vi "LC_Read_Number.vi"(8 "Cutted Sample Sequence":string="TCTAGACTATCTCACTCTCAGATGAGATCGATAGATCAGT", 9 "Level Composition":string[](array[string]), 11 "LSPX_C2":T1) -> (3 "Assigned#_CL":T2)   [LabVIEW 2018]
panel:
  out "Tri_MxRight#":i32[](array[numeric])
  out "Di_MxRight#":i32[](array[numeric])
  out "Mono_MxRight#":i32[](array[numeric])
  out "Tri_Assigned#":i32[](array[numeric])
  out "Di_Assigned#":i32[](array[numeric])
  out "Mono_Assigned#":i32[](array[numeric])
  out "MxRight_Array":string[](array[string])
  out "Assigned_Array":string[](array[string])
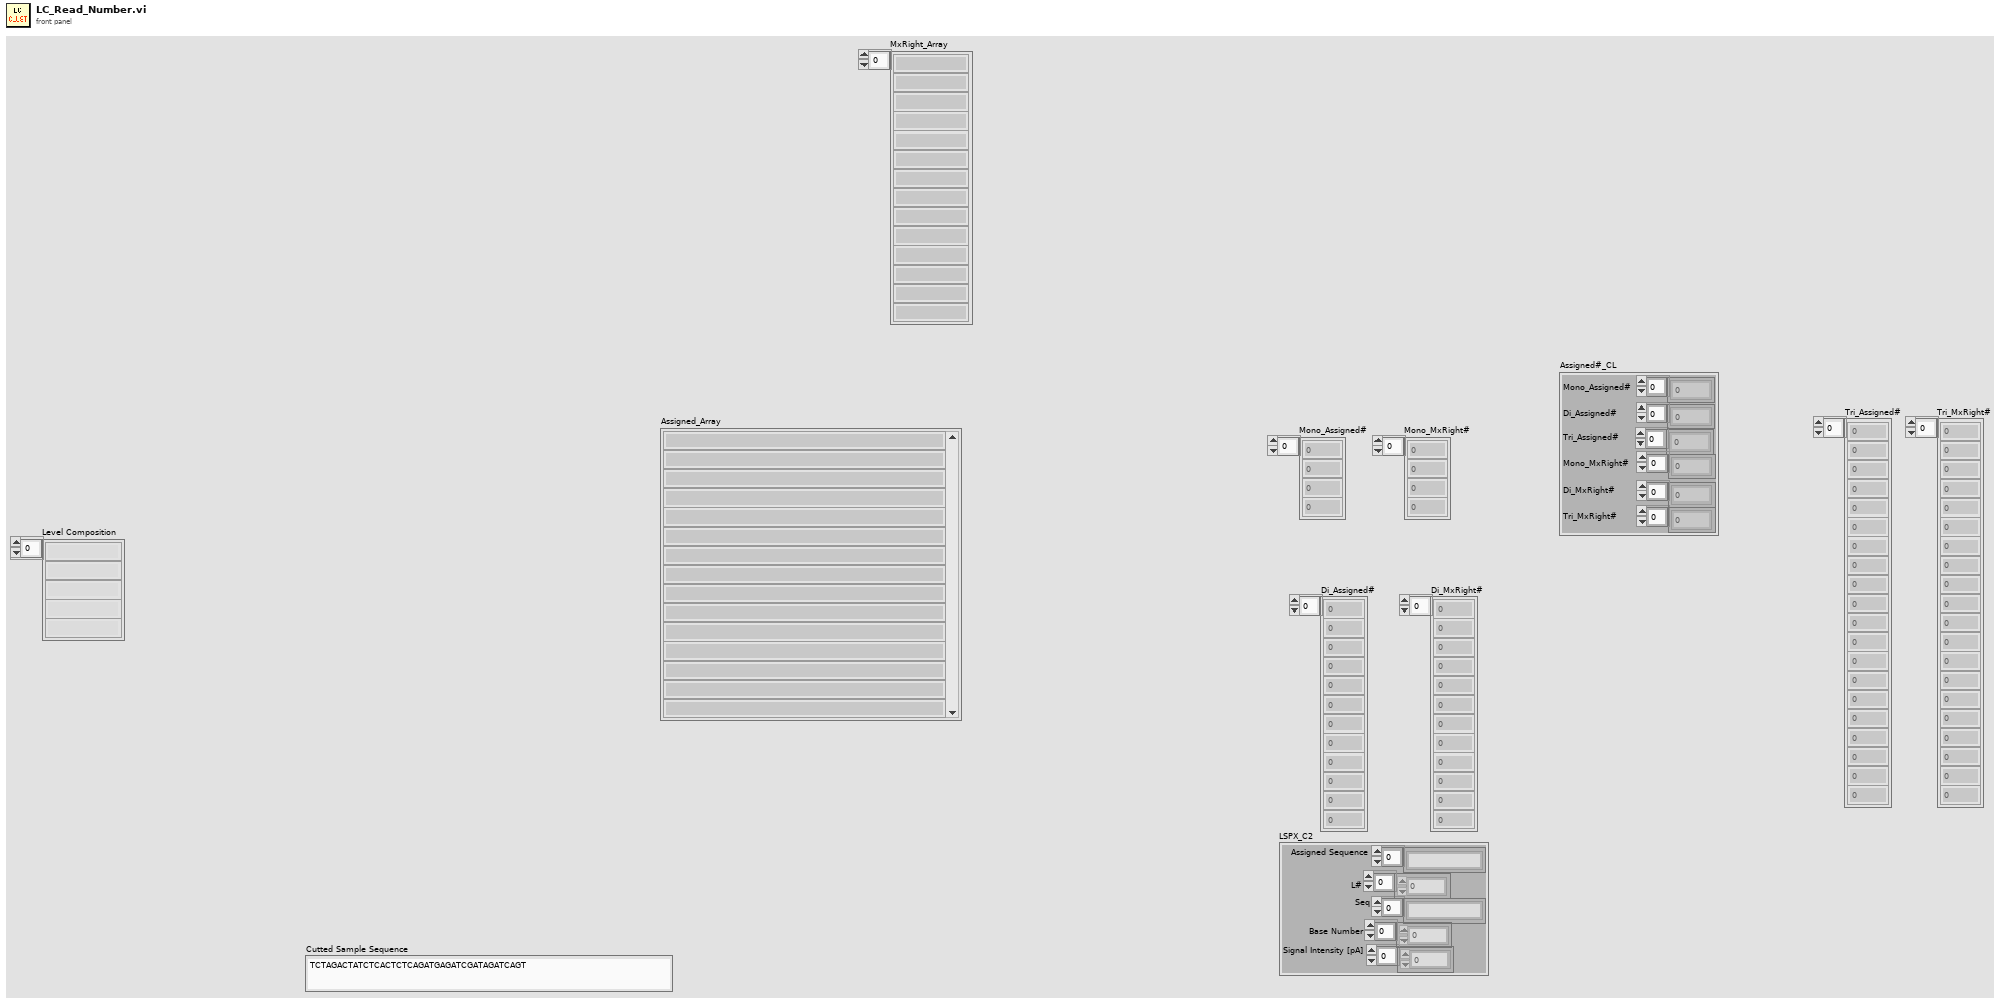
[diagram p1: front panel]
types:
  T1 = cluster{"Assigned Sequence":string[], "L#":i32[], "Seq":string[], "Base Number":i32[], "Signal Intensity [pA]":dbl[]}
  T2 = cluster{"Mono_Assigned#":i32[], "Di_Assigned#":i32[], "Tri_Assigned#":i32[], "Tri_MxRight#":i32[], "Di_MxRight#":i32[], "Mono_MxRight#":i32[]}
  T3 = cluster{"MonoBase_Array_Tag":string[], "DiBase_Array_Tag":string[], "TriBase_Array_Tag":string[]}
  T4 = cluster{i32[], i32[], i32[], i32[], i32[], i32[]}
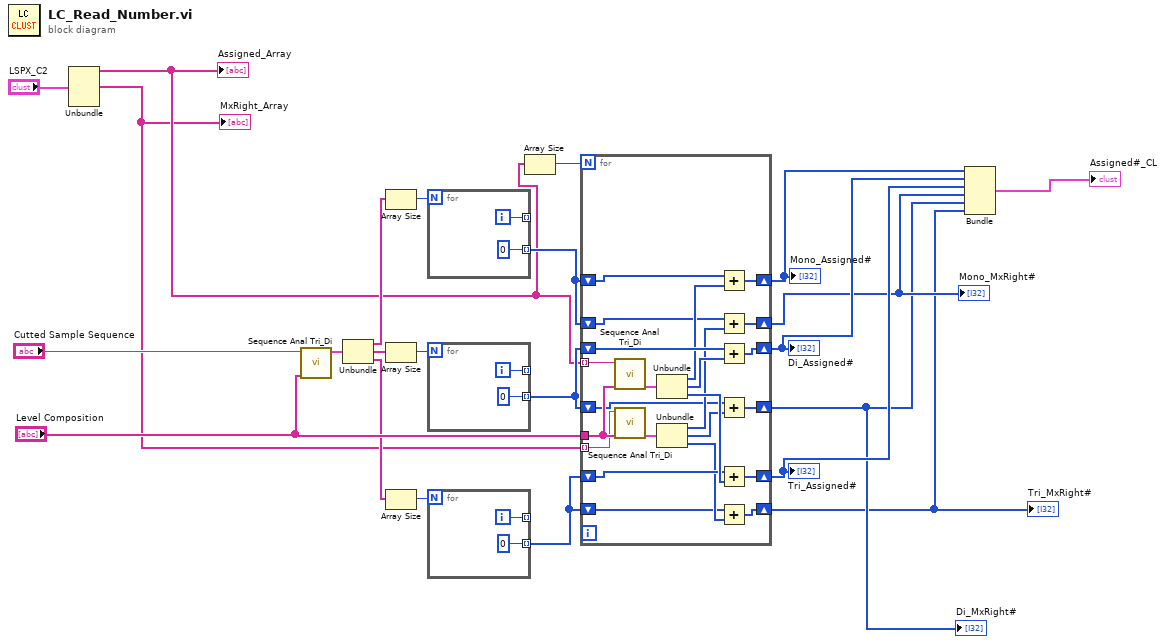
[diagram p0: block diagram]
diagram:
  n1 = Unbundle("LSPX_C2") -> ("Assigned Sequence"=w5:string[], "Seq"=w4:string[])  [unwired: 3 out]
  "Assigned_Array" <- w5
  "MxRight_Array" <- w4
  n2 = call "Sequence Anal Tri_Di.vi"("Level Composition"="Level Composition", "String"="Cutted Sample Sequence") -> ("Base Tag"=w22:T3)  [unwired: 7 in, 2 out]
  n3 = Unbundle(w22) -> ("MonoBase_Array_Tag"=w11:string[], "DiBase_Array_Tag"=w13:string[], "TriBase_Array_Tag"=w12:string[])
  n4 = Array Size(array=w11) -> (size(s)=w20:i32)
  n5 = Array Size(array=w13) -> (size(s)=w19:i32)
  n6 = Array Size(array=w12) -> (size(s)=w18:i32)
  n7 = for {
    N: w20 -> [_]
    tunnel: [0 ("index")] -> w17 mode=indexing
    tunnel: [w24] -> _ mode=indexing
    i -> [w24]
  }
  n8 = for {
    N: w19 -> [_]
    tunnel: [0 ("index")] -> w16 mode=indexing
    tunnel: [w26] -> _ mode=indexing
    i -> [w26]
  }
  n9 = for {
    N: w18 -> [_]
    tunnel: [0 ("index")] -> w15 mode=indexing
    tunnel: [w28] -> _ mode=indexing
    i -> [w28]
  }
  n10 = Array Size(array=w5) -> (size(s)=w14:i32)
  n11 = for {
    N: w14 -> [_]
    tunnel: w4 -> [w30] mode=indexing
    tunnel: "Level Composition" -> [w42]
    shift-right: [w51] -> w10
    shift-left: w17 -> [w50]
    shift-right: [w47] -> w8
    shift-left: w15 -> [w46]
    shift-right: [w45] -> w9
    shift-left: w16 -> [w44]
    shift-right: [w37] -> w3
    shift-left: w17 -> [w32]
    shift-right: [w36] -> w2
    shift-left: w16 -> [w33]
    shift-right: [w35] -> w1
    shift-left: w15 -> [w34]
    tunnel: w5 -> [w31] mode=indexing
    n12 = call "Sequence Anal Tri_Di.vi"("Level Composition"=w42, "String"=w31) -> ("BaseNumber"=w52:cluster{i32[], i32[], i32[]})  [unwired: 7 in, 2 out]
    n13 = call "Sequence Anal Tri_Di.vi"("Level Composition"=w42, "String"=w30) -> ("BaseNumber"=w41:cluster{i32[], i32[], i32[]})  [unwired: 7 in, 2 out]
    n14 = Unbundle(w52) -> (w43:i32[], w49:i32[], w48:i32[])
    n15 = Unbundle(w41) -> (w40:i32[], w39:i32[], w38:i32[])
    n16 = Add(x=w50, y=w43) -> (x+y=w51:i32[])
    n17 = Add(x=w32, y=w40) -> (x+y=w37:i32[])
    n18 = Add(x=w44, y=w49) -> (x+y=w45:i32[])
    n19 = Add(x=w33, y=w39) -> (x+y=w36:i32[])
    n20 = Add(x=w46, y=w48) -> (x+y=w47:i32[])
    n21 = Add(x=w34, y=w38) -> (x+y=w35:i32[])
  }
  "Mono_Assigned#" <- w10
  "Di_Assigned#" <- w9
  "Tri_Assigned#" <- w8
  "Mono_MxRight#" <- w3
  "Di_MxRight#" <- w2
  "Tri_MxRight#" <- w1
  n22 = Bundle(w10, w9, w8, w3, w2, w1) -> (→"Assigned#_CL":T4)  [unwired: 1 in]
